vi "Generate filler images.vi"(8 "error in (no error)":errorcluster) -> (0 "error out":errorcluster)   [LabVIEW 2020, in "DAQ Timed SPIM.lvlib" / "HamamatsuFluor_v2.lvlib"]
uses:
  HamamatsuFluor_v2.lvlib
  <vilib>/vision/NI_Vision_Development_Module.lvlib
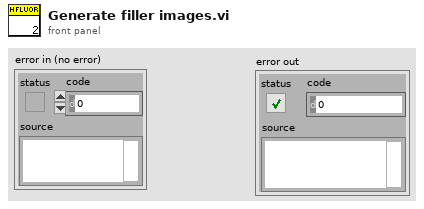
[diagram p1: front panel]
types:
  T1 = typedef "Image Type" = u32
  T2 = typedef "IMAQ Image.ctl" = refnum<image>
  T3 = cluster{"Desired Font (Application)":enum16{"User-specified Font", "Application Font", "System Font", "Dialog Font"}, "[User-specified Font]":cluster{"Font Name":string, "Size":i16, "Strikeout?":bool, "Italic?":bool, "Underline?":bool, "Outline?":bool, "Shadow?":bool, "Bold?":bool, "Rotation Angle":dbl}, "Horizontal Alignment":i16, "Vertical Alignment":i16}
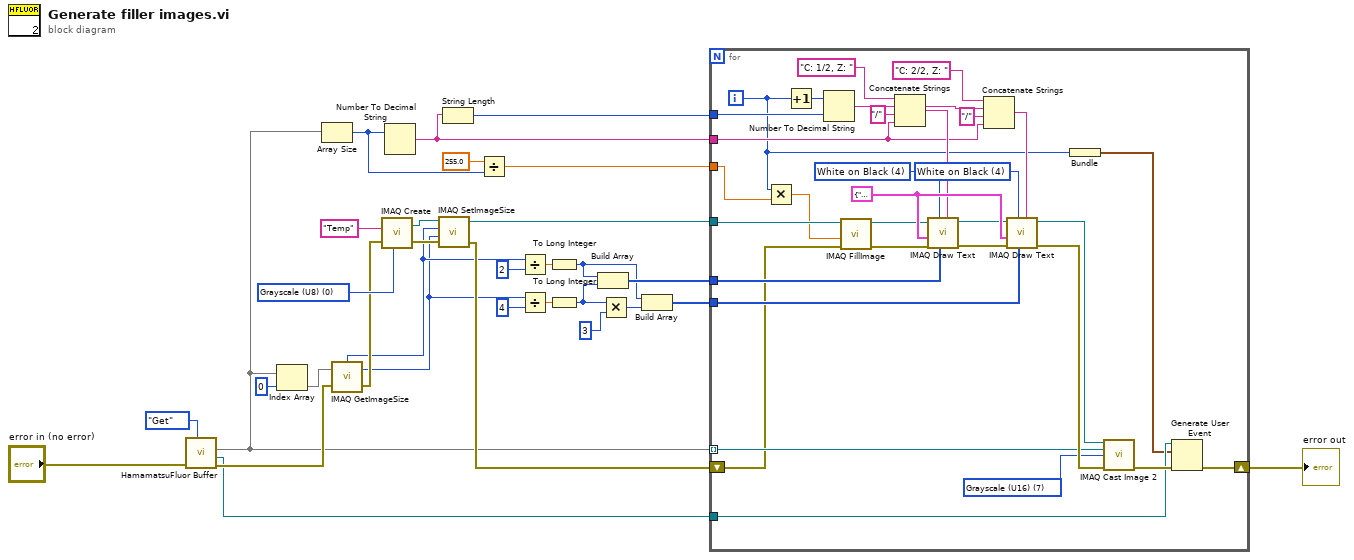
[diagram p0: block diagram]
diagram:
  w31 = T1 0 items=["Grayscale (U8)", "Grayscale (I16)", "Grayscale (SGL)", "Complex (CSG)", "RGB (U32)", "HSL (U32)", "RGB (U64)", "Grayscale (U16)"] ("Image Type")
  n1 = call "HamamatsuFluor Buffer.vi"("Action"=enum16{"Get", "Acquire", "Release"}."Get", "error in (no error)"="error in (no error)") -> ("error out"=w22:errorcluster, "Buffer Write Event"=w4:refnum<user-event>, 2:w20)  [unwired: 6 in, 1 out]
  n2 = Index Array(array=w20, index=0) -> (element=w24)
  n3 = Array Size(array=w20) -> (size(s)=w2:i32)
  n4 = call "IMAQ GetImageSize"("Image"=w24, "error in (no error)"=w22) -> ("Y Resolution"=w7:i32, "X Resolution"=w8:i32, "error out"=w23:errorcluster)  [unwired: 2 in]
  n5 = call "IMAQ Create"("Image Name"="Temp", "Image Type"=w31, "error in (no error)"=w23) -> ("New Image"=w29:T2, "error out"=w30:errorcluster)  [unwired: 2 in]
  n6 = Number To Decimal String(number=w2) -> (decimal integer string=w19:string)  [unwired: 1 in]
  n7 = call "IMAQ SetImageSize"("error in (no error)"=w30, "Y Resolution"=w7, "X Resolution"=w8, "Image"=w29) -> ("error out"=w28:errorcluster, "Image Out"=w21:T2)  [unwired: 1 in]
  n8 = String Length(string=w19) -> (length=w18:i32)
  n9 = Divide(x=255.0, y=w2) -> (x/y=w1:dbl)
  n10 = Divide(x=w8, y=2) -> (x/y=w15:dbl)
  n11 = Divide(x=w7, y=4) -> (x/y=w16:dbl)
  n12 = To Long Integer(number=w15) -> (32bit integer=w6:i32)
  n13 = To Long Integer(number=w16) -> (32bit integer=w17:i32)
  n14 = Build Array(w6, w17) -> (w11:i32[])
  n15 = Multiply(x=w17, y=3) -> (x*y=w10:i32)
  n16 = Build Array(w6, w10) -> (w9:i32[])
  n17 = for {
    shift-right: [w42] -> w27
    shift-left: w28 -> [w39]
    tunnel: w21 -> [w36]
    tunnel: w20 -> [w45] mode=indexing
    tunnel: w19 -> [w49]
    tunnel: w18 -> [w48]
    tunnel: w11 -> [w47]
    tunnel: w9 -> [w46]
    tunnel: w4 -> [w41]
    tunnel: w1 -> [w35]
    i -> [w34]
    w44 = T1 7 items=["Grayscale (U8)", "Grayscale (I16)", "Grayscale (SGL)", "Complex (CSG)", "RGB (U32)", "HSL (U32)", "RGB (U64)", "Grayscale (U16)"] ("Image Type")
    w61 = 4 items=["White", "Black", "Inverted", "Black on White", "White on Black"] ("Color")
    w62 = 4 items=["White", "Black", "Inverted", "Black on White", "White on Black"] ("Color")
    w64 = T3 {"Desired Font (Application)"=enum."User-specified Font", "[User-specified Font]"={"Font Name"="", "Size"=48, "Strikeout?"=FALSE, "Italic?"=FALSE, "Underline?"=FALSE, "Outline?"=FALSE, "Shadow?"=FALSE, "Bold?"=TRUE, "Rotation Angle"=0.0}, "Horizontal Alignment"=1, "Vertical Alignment"=0} ("Font, Size & Style")
    n18 = Multiply(x=w34, y=w35) -> (x*y=w33:dbl)
    n19 = Increment(x=w34) -> (x+1=w56:i32)
    n20 = Number To Decimal String(number=w56, width (-)=w48) -> (decimal integer string=w54:string)
    n21 = call "IMAQ FillImage"("error in (no error)"=w39, "Pixel Value (U8, U16, I16, Float)"=w33, "Image"=w36) -> ("error out"=w38:errorcluster, "Image Out"=w37:T2)  [unwired: 7 in]
    n22 = Concatenate Strings("C: 1/2, Z: " ("string"), w54, "/" ("string"), w49) -> (w51:string)
    n23 = call "IMAQ Draw Text"("String"=w51, "Insertion Point"=w47, "Color"=w62, "error in (no error)"=w38, "Font, Size & Style"=w64, "Image Src"=w37) -> ("error out"=w58:errorcluster, "Image Dst Out"=w63:T2)  [unwired: 2 in, 2 out]
    n24 = Concatenate Strings("C: 2/2, Z: " ("string"), w54, "/" ("string"), w49) -> (w50:string)
    n25 = call "IMAQ Draw Text"("String"=w50, "Insertion Point"=w46, "Color"=w61, "error in (no error)"=w58, "Font, Size & Style"=w64, "Image Src"=w63) -> ("error out"=w60:errorcluster, "Image Dst Out"=w59:T2)  [unwired: 2 in, 2 out]
    n26 = Bundle(w34) -> (w40:cluster{i32})  [unwired: 1 in]
    n27 = call "IMAQ Cast Image 2"("Image Src"=w59, "Image Dst"=w45, "Image Type"=w44, "error in (no error)"=w60) -> ("error out"=w43:errorcluster)  [unwired: 10 in, 1 out]
    n28 = Generate User Event(user event=w41, event data cluster=w40, error in=w43) -> (error out=w42:errorcluster)  [unwired: 1 in, 1 out]
  }
  "error out" <- w27
